vi "Test_Full_Run_2.vi"(8 "error in":errorcluster, 10 "Run Wait ms":i32=40000, 11 "Sequence Path":path=path "C:/Users/DynaAdmin/PycharmProjects/Universal-sequence-executor-AF/configs/sequences/vtu_actual_sequence.json") -> (0 "error out":errorcluster)   [LabVIEW 2026]
doc: "Full run with PROPER dataflow: Launch -> Load -> [2s wait in a While Loop tunnelling the error] -> Start -> [40s wait] -> Normal Stop -> notify, ONE error wire through all. Evidence: traces + results CSV."
uses:
  src/Executor/Sequence Executor.lvclass
  src/Executor Messages/Load Sequence Msg/Load Sequence Msg.lvclass/Load Sequence Msg.ctl
  <vilib>/ActorFramework/Message Enqueuer/Message Enqueuer.lvclass/Message Enqueuer.ctl
  <vilib>/ActorFramework/Message Enqueuer/Enqueue.vi
  src/Executor Messages/Load Sequence Msg/Load Sequence Msg.lvclass
  src/Executor Messages/Start Sequence Msg/Start Sequence Msg.lvclass
  <vilib>/ActorFramework/Stop Msg/Stop Msg.lvclass
  <vilib>/ActorFramework/Message Priority Queue/Priority Enqueue.vi
  <vilib>/ActorFramework/Actor/Actor.lvclass
panel:
  out "Start error":errorcluster
  out "Load error":errorcluster
  out "Stopped cleanly":bool
  out "Feedback Chart":dbl
  out "Verdict":string
  out "Channel Values":string[][](array[string])
  out "Step Table":string[][](array[string])
  out "Step Index":i32
  out "Status":string
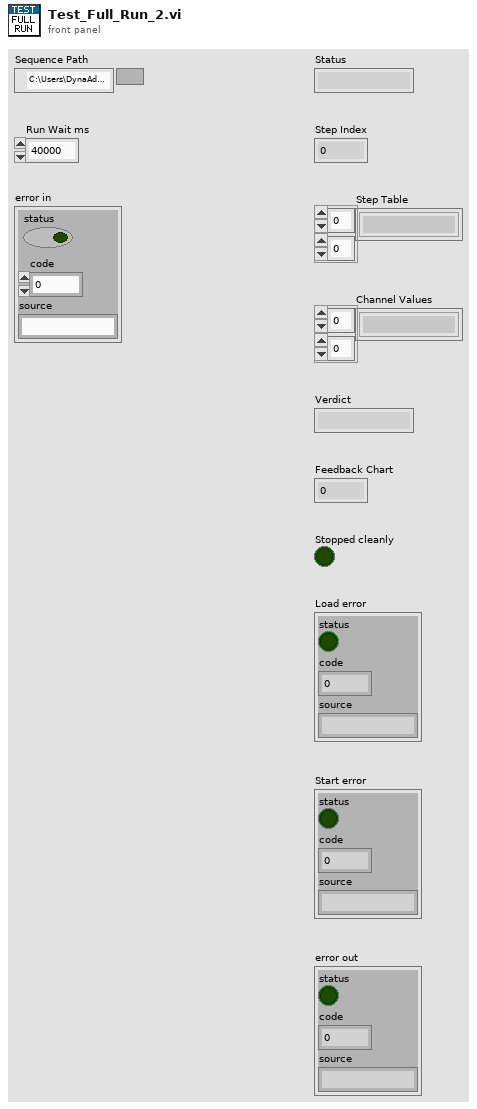
[diagram p1: front panel]
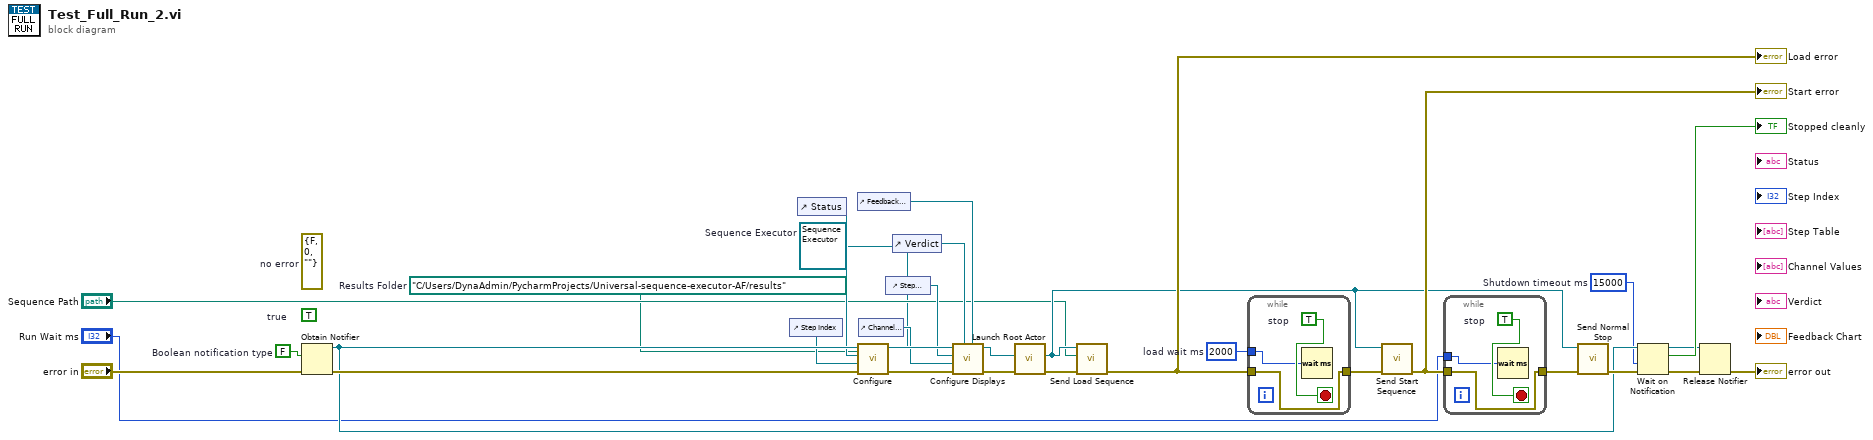
[diagram p0: block diagram]
diagram:
  w5 = 2000  # load wait ms
  (unwired) TRUE  # true
  w4 = path "C:/Users/DynaAdmin/PycharmProjects/Universal-sequence-executor-AF/results"  # Results Folder
  w3 = 15000  # Shutdown timeout ms
  (unwired) errorcluster {"status"=FALSE, "code"=0, "source"=""}  # no error
  w2 = FALSE  # Boolean notification type
  w1 = refnum<class "Sequence Executor.lvclass"> refnum  # Sequence Executor
  n1 = Obtain Notifier(notification data type=w2, error in (no error)="error in") -> (notifier out=w15:refnum<notifier>, error out=w16:errorcluster)  [unwired: 2 in, 1 out]
  n2 = control-ref of="Step Index"() -> (w10:refnum<vi>)
  n3 = control-ref of="Status"() -> (w9:refnum<vi>)
  n4 = control-ref of="Feedback Chart"() -> (w14:refnum<vi>)
  n5 = call "Configure.vi"("Results Folder"=w4, "Stopped Notification"=w15, "error in"=w16, "Step Index Display"=w10, "Status Display"=w9, "Sequence Executor in"=w1) -> ("error out"=w18:errorcluster, "Sequence Executor out"=w17:refnum<class "Sequence Executor.lvclass">)  [unwired: 4 in]
  n6 = control-ref of="Channel Values"() -> (w12:refnum<vi>)
  n7 = control-ref of="Step Table"() -> (w11:refnum<vi>)
  n8 = control-ref of="Verdict"() -> (w13:refnum<vi>)
  n9 = call "Configure Displays.vi"("Feedback Chart"=w14, "Verdict Display"=w13, "error in"=w18, "Channel Values Display"=w12, "Step Table Display"=w11, "Sequence Executor in"=w17) -> ("error out"=w20:errorcluster, "Sequence Executor out"=w19:refnum<class "Sequence Executor.lvclass">)  [unwired: 4 in]
  n10 = call <vilib>:"Launch Root Actor.vi"("error in (no error)"=w20, "Actor"=w19) -> ("error out"=w22:errorcluster, "Actor's Enqueuer"=w21:refnum<class "Message Enqueuer.lvclass">)  [unwired: 8 in]
  n11 = call "Send Load Sequence.vi"("error in (no error)"=w22, "path"="Sequence Path", "Message Enqueuer"=w21) -> ("error out"=w23:errorcluster)  [unwired: 7 in, 1 out]
  "Load error" <- w23
  n12 = while {
    tunnel: w5 -> [w33]
    tunnel: w23 -> [w32]
    tunnel: [w32] -> w24
    stop <- w34 stop-if-true
    w34 = TRUE  # stop
    n13 = Wait (ms)(milliseconds to wait=w33) -> ()  [unwired: 1 out]
  }
  n14 = call "Send Start Sequence.vi"("error in (no error)"=w24, "Message Enqueuer"=w21) -> ("error out"=w25:errorcluster)  [unwired: 8 in, 1 out]
  "Start error" <- w25
  n15 = while {
    tunnel: "Run Wait ms" -> [w36]
    tunnel: w25 -> [w35]
    tunnel: [w35] -> w26
    stop <- w37 stop-if-true
    w37 = TRUE  # stop
    n16 = Wait (ms)(milliseconds to wait=w36) -> ()  [unwired: 1 out]
  }
  n17 = call <vilib>:"Send Normal Stop.vi"("error in (no error)"=w26, "Message Enqueuer"=w21) -> ("error out"=w27:errorcluster)  [unwired: 9 in]
  n18 = Wait on Notification(notifier=w15, timeout in ms (-1)=w3, error in (no error)=w27) -> (notifier out=w28:refnum<notifier>, notification=→"Stopped cleanly":bool, error out=w30:errorcluster)  [unwired: 1 in, 1 out]
  n19 = Release Notifier(notifier=w28, error in (no error)=w30) -> (error out=→"error out":errorcluster)  [unwired: 1 in, 2 out]
